vi "Handle Activation.vi"(8 "error in (no error)":errorcluster, 10 "Activation":T1, 11 "UserEventActivationHandler in":refnum<class "UserEventActivationHandler.lvclass">) -> ()   [LabVIEW 2026, in "ToastNotification.lvlib" / "UserEventActivationHandler.lvclass"]
doc: "Dynamic-dispatch extension point for an injected activation handler. Override this method in a child class to process Activation.Arguments and Activation.User Inputs. The current base implementation performs no action and propagates the incoming error; it displays no dialog. Protocol-activation buttons are handled by Windows rather than this method. Application handlers should return promptly and send long-running work to a caller-owned queue or user event. Never close the service from its callback."
uses:
  UserEventActivationHandler.lvclass
  ToastNotification/Activation.ctl
  ToastNotification/Argument.ctl
  Activation Event Data.ctl
  UserEventActivationHandler.lvclass/UserEventActivationHandler.ctl
  Read Event Ref.vi
  ToastNotification/ToastNotification.lvlib
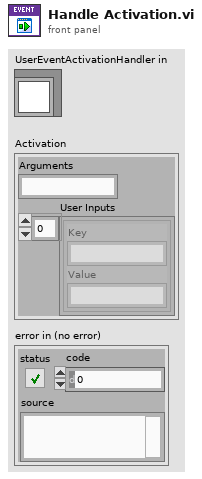
[diagram p1: front panel]
types:
  T1 = typedef "ToastNotification.lvlib/Activation.ctl" = cluster{"Arguments":string, "User Inputs":T2[]}
  T2 = typedef "ToastNotification.lvlib/Argument.ctl" = cluster{"Key":string, "Value":string}
  T3 = typedef "ToastNotification.lvlib/UserEventActivationHandler.lvclass/Activation Event Data.ctl" = cluster{"Activation":T1, "error":errorcluster}
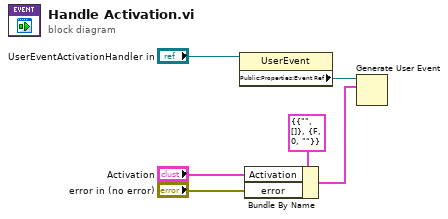
[diagram p0: block diagram]
diagram:
  n1 = property class="UserEvent"(reference="UserEventActivationHandler in") -> ("Public:Properties:Event Ref"=w5:refnum<user-event>)  [unwired: 1 in, 2 out]
  n2 = Bundle By Name(cluster=T3 {"Activation"={"Arguments"="", "User Inputs"=[]}, "error"={"status"=FALSE, "code"=0, "source"=""}} ("event data"), "Activation"="Activation", "error"="error in (no error)") -> (w3:T3)
  n3 = Generate User Event(user event=w5, event data cluster=w3) -> ()  [unwired: 2 in, 2 out]
